vi "Data_Connect.vi"(8 "error in (no error)":errorcluster) -> (0 "error out":errorcluster, 2 "Enum":T1, 3 "writer endpoint":refnum<k21>)   [LabVIEW 2025]
uses:
  states.ctl
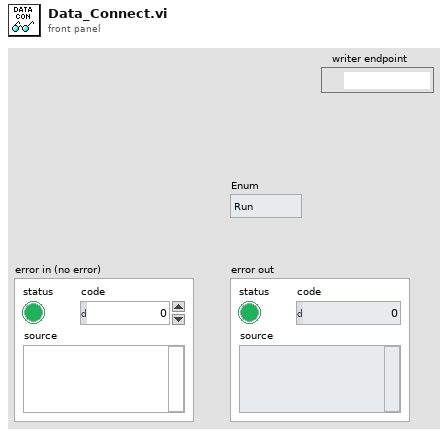
[diagram p1: front panel]
types:
  T1 = typedef "states.ctl" = enum16{"Run", "Connect"}
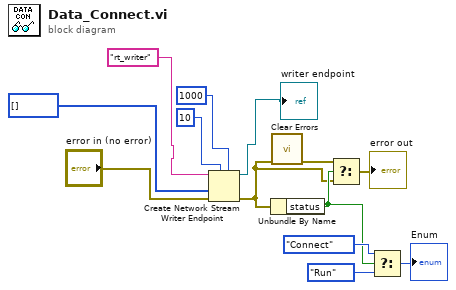
[diagram p0: block diagram]
diagram:
  n1 = Create Network Stream Writer Endpoint(5:1000 ("timeout in ms (-1)"), 7:10 ("reader buffer size"), 8:"error in (no error)", 9:i16[] [], 11:"rt_writer" ("reader name")) -> (0:w2:errorcluster, 3:→"writer endpoint":refnum<k21>)  [unwired: 2 in]
  n2 = Unbundle By Name(w2) -> ("status"=w9:bool)
  n3 = call <vilib>:"Clear Errors.vi"("error in (no error)"=w2) -> ("error out"=w8:errorcluster)  [unwired: 5 in, 1 out]
  n4 = Select(t=w8, s=w9, f=w2) -> (s? t:f=→"error out":errorcluster)
  n5 = Select(t=states."Connect", s=w9, f=states."Run") -> (s? t:f=→"Enum":T1)
